vi "NR set Modulation Table.vi"(8 "error in (no error)":errorcluster caption="에러 입력(에러 없음)", 11 "Instrument Manager 입력":refnum<class "Instrument Manager.lvclass">) -> (0 "error out":errorcluster caption="에러 출력", 3 "Instrument Manager 출력":refnum<class "Instrument Manager.lvclass">)   [LabVIEW 2023, in "Instrument Manager.lvclass"]
uses:
  Instrument Manager.lvclass
  Instrument Manager.lvclass/Instrument Manager.ctl
  Module/ANRITSU Call Box/Type Definition/Uplink Downlink Enum.ctl
  Module/ANRITSU Call Box/ANRITSU Call Box.lvlib
  Module/ANRITSU Call Box/Type Definition/Modulation Table Selector.ctl
  Module/ANRITSU Call Box/Interface Class/Anritsu Call Box.lvclass
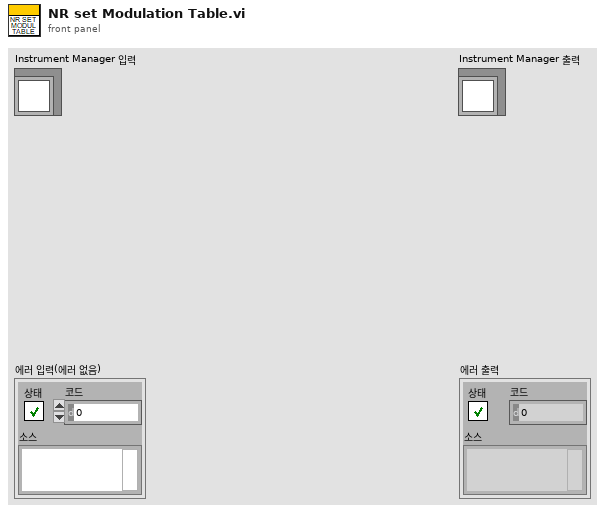
[diagram p1: front panel]
types:
  T1 = typedef "ANRITSU Call Box.lvlib/Modulation Table Selector.ctl" = enum16{"64QAM Table", "256QAM Table"}
  T2 = typedef "ANRITSU Call Box.lvlib/Uplink Downlink Enum.ctl" = enum16{"Uplink", "Downlink"}
  T3 = cluster{"Anritsu Call Box":refnum<class "Anritsu Call Box.lvclass">, "Spectrum Analyzer":refnum<class "Interface_Spectrum.lvclass">, "RF Switch Box":refnum<class "RF Filter Box.lvclass">, "Turn Table":refnum<class "Interface - Turn Table.lvclass">, "Mast":refnum<class "Interface - Mast.lvclass">, "3D Controller":refnum<class "Interface_3D Controller.lvclass">}
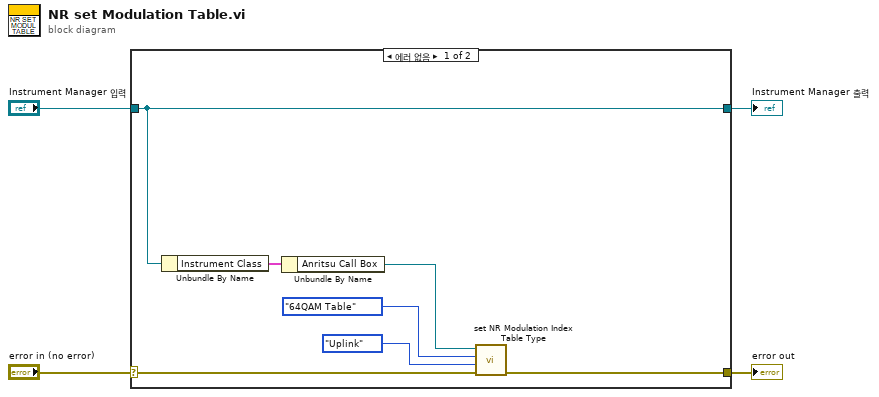
[diagram p0: block diagram]
diagram:
  n1 = case shown="에러 없음" "error in (no error)" {
    selector: "error in (no error)" -> [w10 w13]
    tunnel: [w5 w13] -> w3
    tunnel: [w11 w12] -> w1
    tunnel: "Instrument Manager 입력" -> [w11 w12]
    frame No Error {
      n2 = Unbundle By Name(w11) -> ("Instrument Class"=w9:T3)
      n3 = Unbundle By Name(w9) -> ("Anritsu Call Box"=w8:refnum<class "Anritsu Call Box.lvclass">)
      n4 = call-dynamic "set NR Modulation Index Table Type.vi"("error in (no error)"=w10, "Direction"=Uplink_Downlink_Enum."Uplink", "Modulation Table"=Modulation_Table_Selector."64QAM Table", "Anritsu Call Box in"=w8) -> ("error out"=w5:errorcluster)  [unwired: 6 in, 1 out]
    }
    frame Error {
    }
  }
  "error out" <- w3
  "Instrument Manager 출력" <- w1
